vi "ERROR.vi"(8 "?":errorcluster) -> (0 "error":errorcluster)   [LabVIEW 2021]
panel:
  in  "Result 3":bool=TRUE
  in  "Button":bool
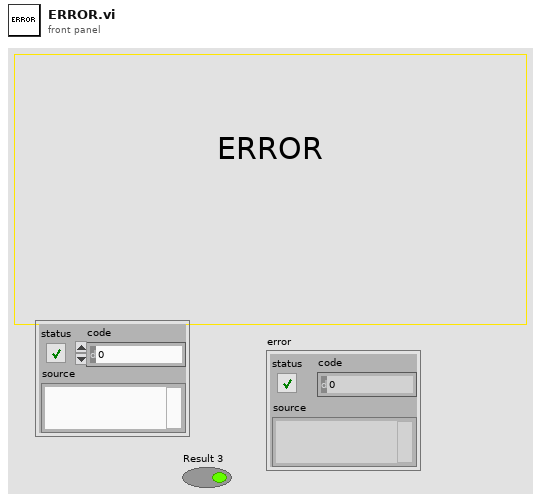
[diagram p1: front panel]
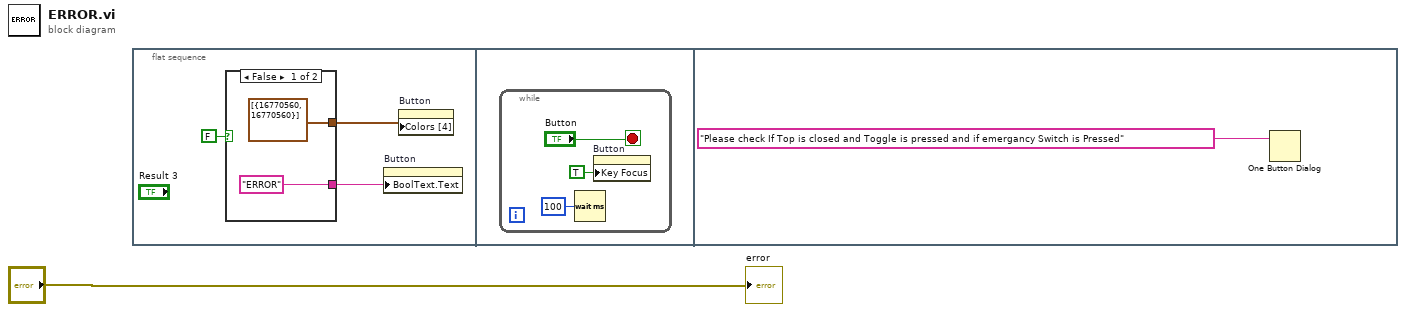
[diagram p0: block diagram]
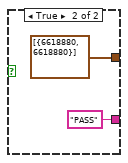
[diagram p2: hidden frame]
diagram:
  n1 = flat-sequence {
    frame #0 {
      n2 = case shown="False" FALSE {
        tunnel: [cluster{u32, u32}[] [{16770560, 16770560}] ("Colors [4]") cluster{u32, u32}[] [{6618880, 6618880}] ("Colors [4]")] -> w4
        tunnel: ["ERROR" ("Boolean Text.Text") "PASS" ("Boolean Text.Text")] -> w3
        frame False {
        }
        frame True {
        }
      }
      n3 = property on="Button" class="Bool"("BoolText.Text"=w3) -> ()  [unwired: 2 in, 2 out]
      n4 = property on="Button" class="Bool"("Colors [4]"=w4) -> ()  [unwired: 2 in, 2 out]
    }
    frame #1 {
      n5 = while {
        stop <- "Button" stop-if-true
        n6 = Wait (ms)(milliseconds to wait=u32 100) -> ()  [unwired: 1 out]
        n7 = property on="Button" class="Bool"("Key Focus"=TRUE) -> ()  [unwired: 2 in, 2 out]
      }
    }
    frame #2 {
      n8 = One Button Dialog(message="Please check If Top is closed and Toggle is pressed and if emergancy Switch is Pressed") -> ()  [unwired: 1 in, 1 out]
    }
  }
  "error" <- "?"
